vi "CIF_Iceoryx_String_Tag Update Test Cases.vi"() -> (0 "error out":errorcluster, 2 "status":string, 3 "pass":bool)   [LabVIEW 2021]
uses:
  CIF_Iceoryx_Chn_String.lvclass
  D:/dev/Packages/CIF_Channels_Core/src/Iceorxy_Channels/CIF_Iceoryx_BB/CIF_Iceoryx_BB.lvclass
  D:/dev/Packages/CIF_Channels_Core/src/CIFChannels/CIFChannels.lvclass
  ChannelCommon/typedef/Direction.ctl
  ChannelCommon/typedef/New FIFO Instance Response.ctl
  CIFChannels/CIFChannels.lvclass/CIFChannels.ctl
  ChannelCommon/typedef/New FIFO Config.ctl
  ChannelCommon/typedef/FIFO Flags.ctl
  ChannelCommon/ChannelCommon.lvlib
  CIFChannels/CIFChannels.lvclass
  <vilib>/CIF Foundation/CIF Iceoryx/Iceoryx.lvlib
  CIF_Iceoryx_BB/CIF_Iceoryx_BB.lvclass
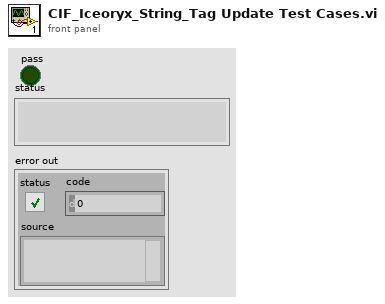
[diagram p1: front panel]
types:
  T1 = typedef "ChannelCommon.lvlib/Direction.ctl" = enum8{"Publisher", "Subscriber"}
  T2 = typedef "ChannelCommon.lvlib/New FIFO Instance Response.ctl" = cluster{"Publisher":string, "Custom Data":u8[]}
  T3 = typedef "ChannelCommon.lvlib/New FIFO Config.ctl" = cluster{"Max Bytes/Msg":u64, "Max Msg/FIFO":u64, "FIFO Flags":T4, "Best Effort Subscribers":u32, "Backpressure Subscribers":u32}
  T4 = typedef "ChannelCommon.lvlib/FIFO Flags.ctl" = cluster{"Backpressure":bool, "Extended Config":bool}
  T5 = typedef "Iceoryx.lvlib/BB Refnum.ctl" = cluster{"refnum":u64, "BB":enum8{"bb"}}
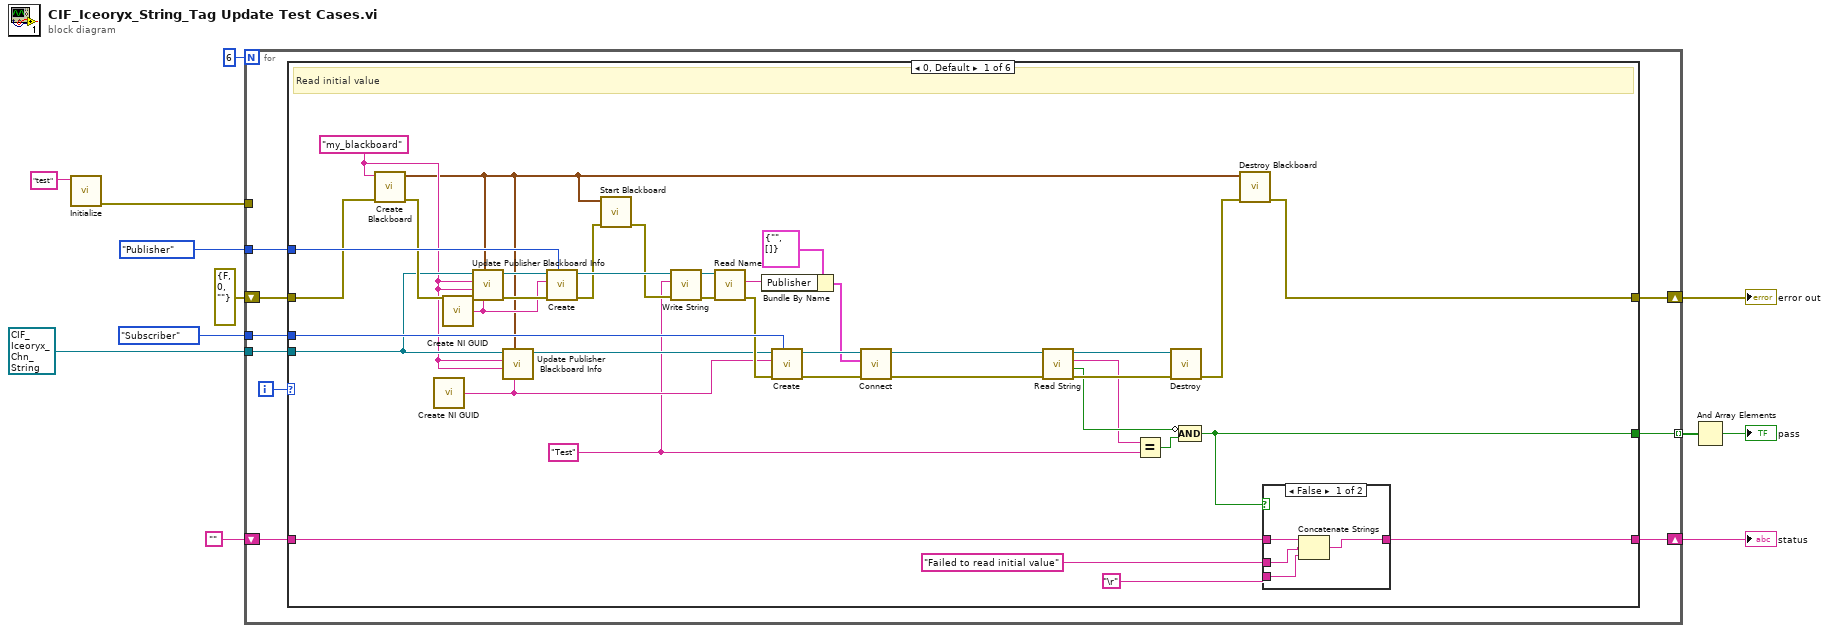
[diagram p0: block diagram]
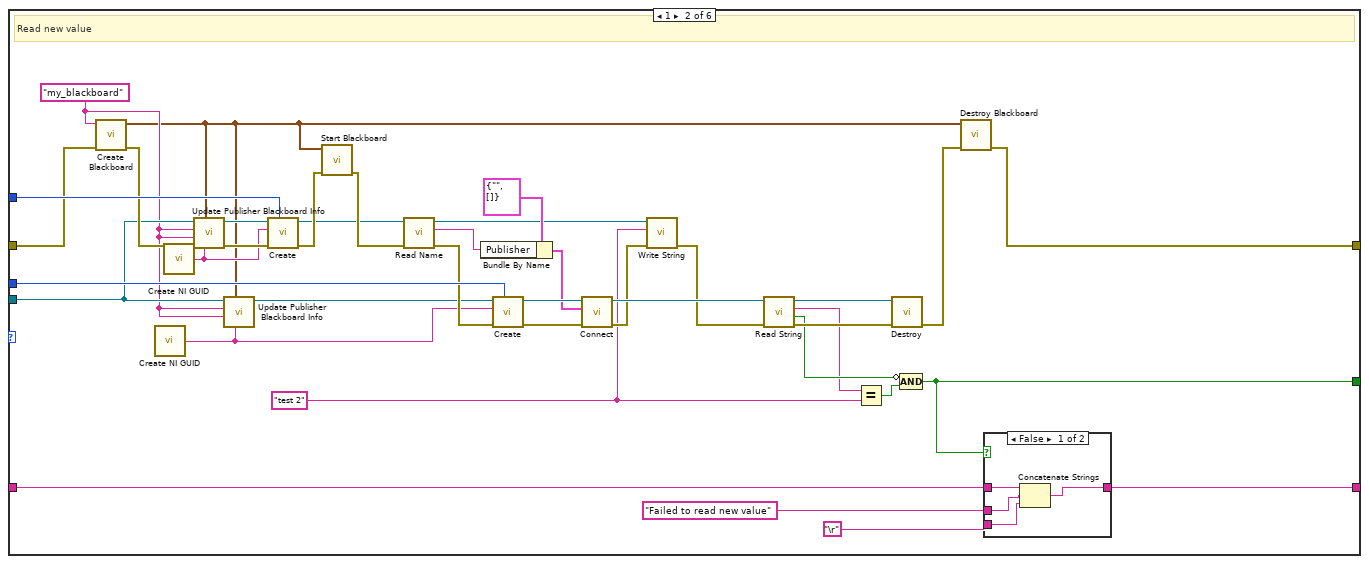
[diagram p3: hidden frame]
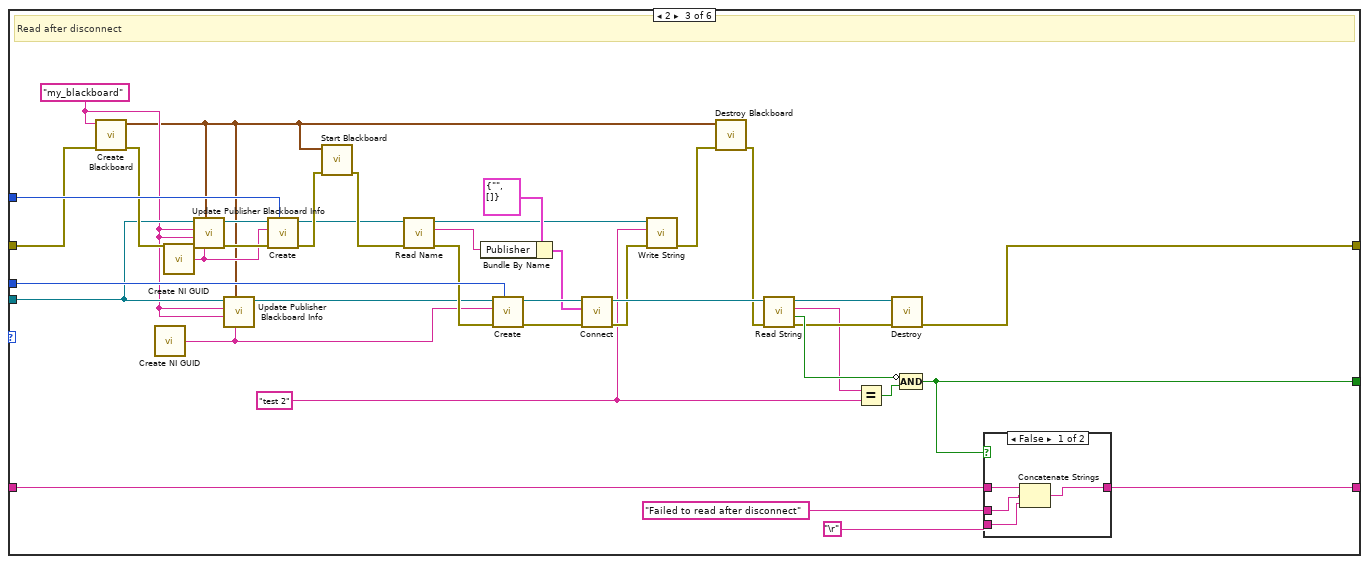
[diagram p5: hidden frame]
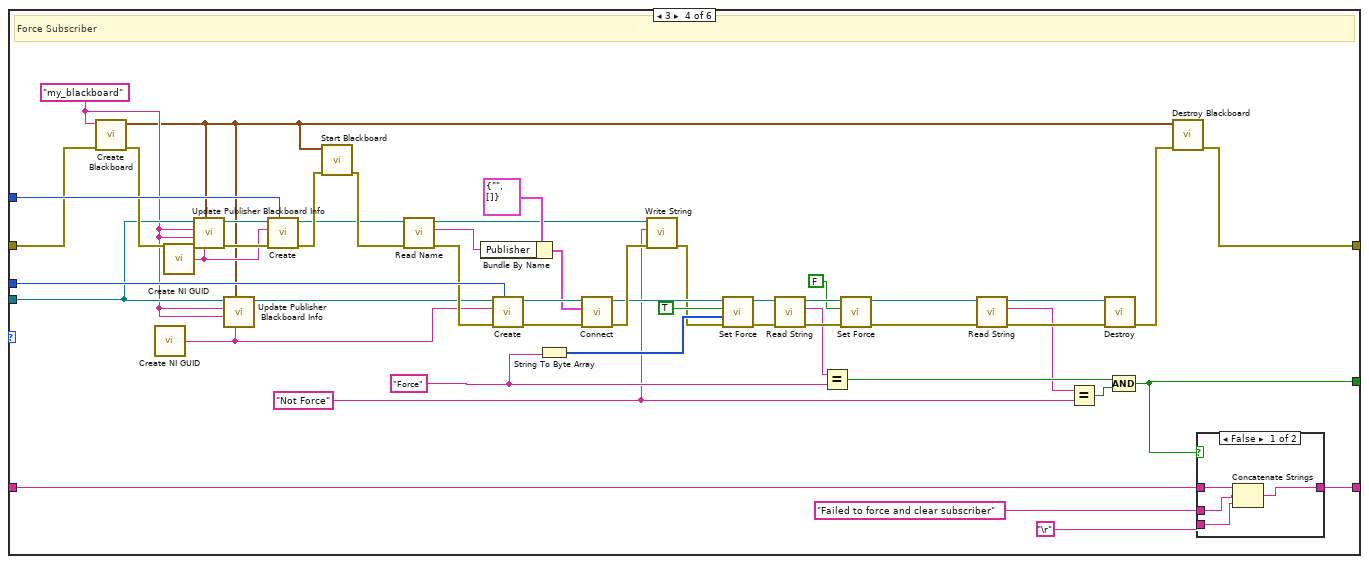
[diagram p7: hidden frame]
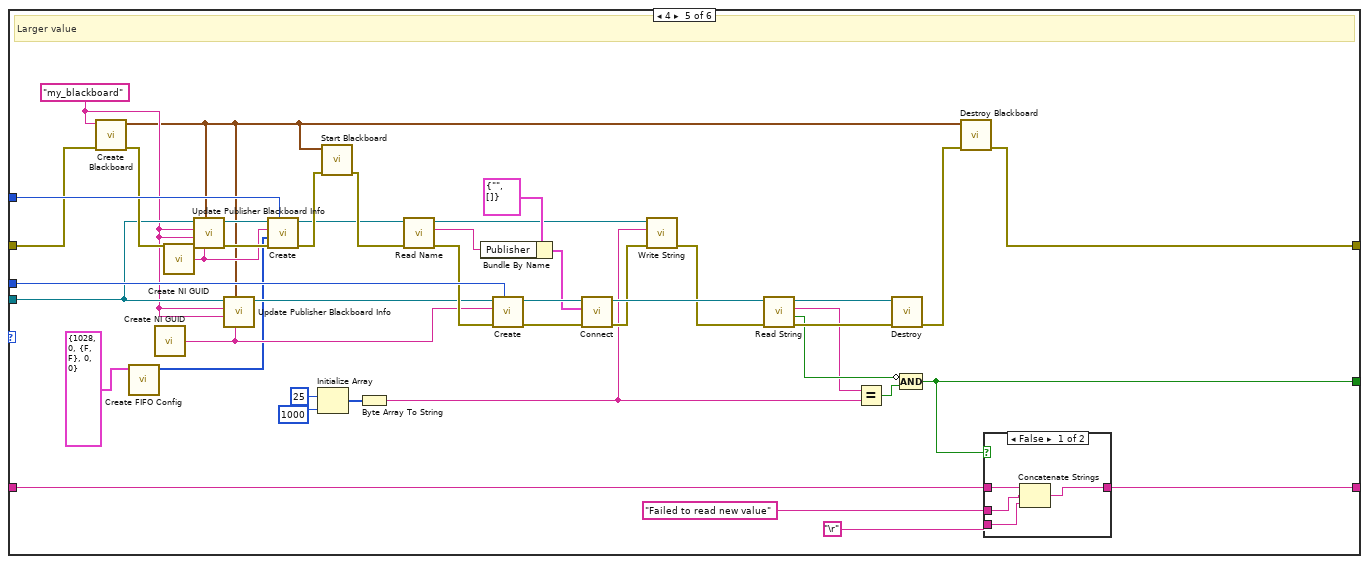
[diagram p9: hidden frame]
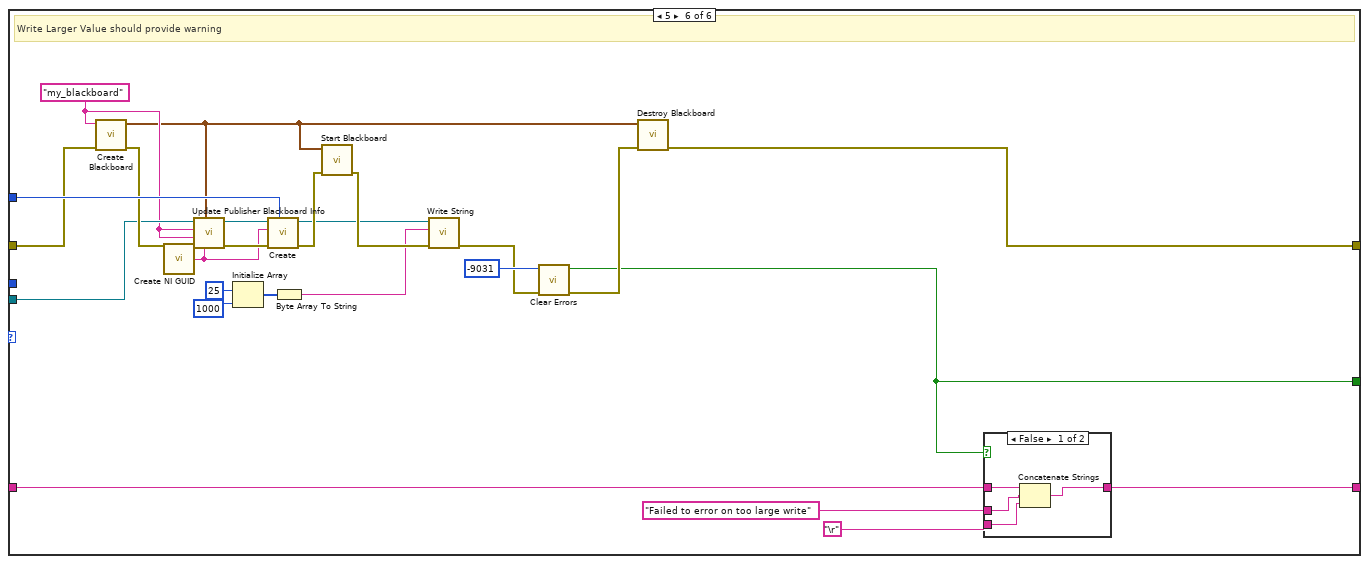
[diagram p11: hidden frame]
diagram:
  n1 = call <vilib>:"Initialize.vi"("Node name"="test") -> ("error out"=w6:errorcluster)  [unwired: 10 in]
  n2 = for {
    N: 6 -> [_]
    tunnel: [w21] -> w12 mode=indexing
    shift-right: [w19] -> w3
    shift-left: errorcluster {"status"=FALSE, "code"=0, "source"=""} ("error out") -> [w20]
    shift-right: [w16] -> w1
    shift-left: "" -> [w17]
    tunnel: refnum<class "CIF_Iceoryx_Chn_String.lvclass"> refnum ("CIF_CIPC_Chn_String.lvclass") -> [w15]
    tunnel: Direction."Publisher" ("Direction") -> [w14]
    tunnel: Direction."Subscriber" ("Direction") -> [w13]
    tunnel: w6 -> [_]
    i -> [w18]
    n3 = case shown="0, Default" w18 {
      tunnel: [w49 w92 w136 w191 w237 w253] -> w21
      tunnel: w20 -> [w42 w86 w130 w186 w231 w272]
      tunnel: [w35 w80 w110 w180 w225 w267] -> w19
      tunnel: w17 -> [w59 w102 w145 w199 w247 w277]
      tunnel: [w58 w101 w144 w198 w246 w276] -> w16
      tunnel: w15 -> [w28 w76 w122 w176 w221 w265]
      tunnel: w14 -> [w47 w90 w134 w190 w235 w273]
      tunnel: w13 -> [w46 w89 w133 w189 w234 _]
      frame 0, Default {
        w23 = "Test"
        w26 = "my_blackboard" ("Blackboard name")
        # "Read initial value"
        n4 = call <vilib>:"Create Blackboard.vi"("error in (no error)"=w42, "Blackboard name"=w26) -> ("error out"=w39:errorcluster, "Blackboard Reference"=w24:T5)  [unwired: 8 in]
        n5 = call <vilib>:"Create NI GUID.vi"() -> ("NI GUID"=w25:string)
        n6 = call <vilib>:"Create NI GUID.vi"() -> ("NI GUID"=w33:string)
        n7 = call "Update Publisher Blackboard Info.vi"("Topic"=w33, "Blackboard Reference"=w24, "error in (no error)"=w39, "Blackboard name"=w26, "Plugin name"=w26, "CIF_Iceoryx_BB in"=w28) -> ("error out"=w38:errorcluster, "CIF_Iceoryx_BB out"=w37:refnum<class "CIF_Iceoryx_Chn_String.lvclass">)  [unwired: 3 in, 1 out]
        n8 = call "Update Publisher Blackboard Info.vi"("Topic"=w25, "Blackboard Reference"=w24, "Blackboard name"=w26, "Plugin name"=w26, "CIF_Iceoryx_BB in"=w28) -> ("CIF_Iceoryx_BB out"=w27:refnum<class "CIF_Iceoryx_Chn_String.lvclass">)  [unwired: 4 in, 2 out]
        n9 = call-dynamic "Create.vi"("Direction"=w47, "error in (no error)"=w38, "Name"=w33, "CIFTag in"=w37) -> ("error out"=w41:errorcluster, "CIFTag out"=w45:refnum<class "CIF_Iceoryx_Chn_String.lvclass">)  [unwired: 6 in]
        n10 = call <vilib>:"Start Blackboard.vi"("error in (no error)"=w41, "Blackboard Reference"=w24) -> ("error out"=w40:errorcluster)  [unwired: 9 in]
        n11 = call-dynamic "Write String.vi"("error in (no error)"=w40, "Data"=w23, "CIFTag in"=w45) -> ("error out"=w32:errorcluster, "CIFTag out"=w31:refnum<class "CIF_Iceoryx_Chn_String.lvclass">)  [unwired: 6 in, 1 out]
        n12 = call "Read Name.vi"("error in (no error)"=w32, "CIFChannels in"=w31) -> ("error out"=w29:errorcluster, "Name"=w30:string)  [unwired: 7 in, 1 out]
        n13 = Bundle By Name(cluster=T2 {"Publisher"="", "Custom Data"=[]} ("Connection"), "Publisher"=w30) -> (w43:T2)
        n14 = call-dynamic "Create.vi"("Direction"=w46, "error in (no error)"=w29, "Name"=w25, "CIFTag in"=w27) -> ("error out"=w54:errorcluster, "CIFTag out"=w55:refnum<class "CIF_Iceoryx_Chn_String.lvclass">)  [unwired: 6 in]
        n15 = call-dynamic "Connect.vi"("error in (no error)"=w54, "Connection"=w43, "CIF_Iceoryx_BB"=w55) -> ("error out"=w34:errorcluster, "CIF_Iceoryx_BB"=w53:refnum<class "CIF_Iceoryx_Chn_String.lvclass">)  [unwired: 7 in]
        n16 = call-dynamic "Read String.vi"("error in (no error)"=w34, "CIFTag in"=w53) -> ("error out"=w51:errorcluster, "timed out?"=w48:bool, "Data"=w22:string, "CIFTag out"=w52:refnum<class "CIF_Iceoryx_Chn_String.lvclass">)  [unwired: 6 in]
        n17 = Equal?(x=w22, y=w23) -> (x = y?=w50:bool)
        n18 = call-dynamic "Destroy.vi"("error in (no error)"=w51, "CIF_Iceoryx_BB in"=w52) -> ("error out"=w36:errorcluster)  [unwired: 8 in, 1 out]
        n19 = Compound Arithmetic op=AND(invert w48, w50) -> (w49:bool)
        n20 = call <vilib>:"Destroy Blackboard.vi"("error in (no error)"=w36, "Blackboard Reference"=w24) -> ("error out"=w35:errorcluster)  [unwired: 8 in, 1 out]
        n21 = case shown="False" w49 {
          tunnel: w59 -> [w63 w64]
          tunnel: [w60 w64] -> w58
          tunnel: "Failed to read initial value" -> [w62 _]
          tunnel: "\r" -> [w61 _]
          frame False {
            n22 = Concatenate Strings(w63, w62, w61) -> (w60:string)
          }
          frame True {
          }
        }
      }
      frame 1 {
        w66 = "test 2" ("Data")
        w74 = "my_blackboard" ("Blackboard name")
        # "Read new value"
        n23 = call <vilib>:"Create Blackboard.vi"("error in (no error)"=w86, "Blackboard name"=w74) -> ("error out"=w84:errorcluster, "Blackboard Reference"=w72:T5)  [unwired: 8 in]
        n24 = call <vilib>:"Create NI GUID.vi"() -> ("NI GUID"=w73:string)
        n25 = call <vilib>:"Create NI GUID.vi"() -> ("NI GUID"=w79:string)
        n26 = call "Update Publisher Blackboard Info.vi"("Topic"=w79, "Blackboard Reference"=w72, "error in (no error)"=w84, "Blackboard name"=w74, "Plugin name"=w74, "CIF_Iceoryx_BB in"=w76) -> ("error out"=w83:errorcluster, "CIF_Iceoryx_BB out"=w82:refnum<class "CIF_Iceoryx_Chn_String.lvclass">)  [unwired: 3 in, 1 out]
        n27 = call "Update Publisher Blackboard Info.vi"("Topic"=w73, "Blackboard Reference"=w72, "Blackboard name"=w74, "Plugin name"=w74, "CIF_Iceoryx_BB in"=w76) -> ("CIF_Iceoryx_BB out"=w75:refnum<class "CIF_Iceoryx_Chn_String.lvclass">)  [unwired: 4 in, 2 out]
        n28 = call-dynamic "Create.vi"("Direction"=w90, "error in (no error)"=w83, "Name"=w79, "CIFTag in"=w82) -> ("error out"=w85:errorcluster, "CIFTag out"=w69:refnum<class "CIF_Iceoryx_Chn_String.lvclass">)  [unwired: 6 in]
        n29 = call <vilib>:"Start Blackboard.vi"("error in (no error)"=w85, "Blackboard Reference"=w72) -> ("error out"=w70:errorcluster)  [unwired: 9 in]
        n30 = call "Read Name.vi"("error in (no error)"=w70, "CIFChannels in"=w69) -> ("error out"=w77:errorcluster, "Name"=w78:string, "CIFChannels out"=w71:refnum<class "CIF_Iceoryx_Chn_String.lvclass">)  [unwired: 7 in]
        n31 = Bundle By Name(cluster=T2 {"Publisher"="", "Custom Data"=[]} ("Connection"), "Publisher"=w78) -> (w87:T2)
        n32 = call-dynamic "Create.vi"("Direction"=w89, "error in (no error)"=w77, "Name"=w73, "CIFTag in"=w75) -> ("error out"=w97:errorcluster, "CIFTag out"=w98:refnum<class "CIF_Iceoryx_Chn_String.lvclass">)  [unwired: 6 in]
        n33 = call-dynamic "Connect.vi"("error in (no error)"=w97, "Connection"=w87, "CIF_Iceoryx_BB"=w98) -> ("error out"=w68:errorcluster, "CIF_Iceoryx_BB"=w96:refnum<class "CIF_Iceoryx_Chn_String.lvclass">)  [unwired: 7 in]
        n34 = call-dynamic "Write String.vi"("error in (no error)"=w68, "Data"=w66, "CIFTag in"=w71) -> ("error out"=w67:errorcluster)  [unwired: 6 in, 2 out]
        n35 = call-dynamic "Read String.vi"("error in (no error)"=w67, "CIFTag in"=w96) -> ("error out"=w94:errorcluster, "timed out?"=w91:bool, "Data"=w65:string, "CIFTag out"=w95:refnum<class "CIF_Iceoryx_Chn_String.lvclass">)  [unwired: 6 in]
        n36 = Equal?(x=w65, y=w66) -> (x = y?=w93:bool)
        n37 = call-dynamic "Destroy.vi"("error in (no error)"=w94, "CIF_Iceoryx_BB in"=w95) -> ("error out"=w81:errorcluster)  [unwired: 8 in, 1 out]
        n38 = Compound Arithmetic op=AND(invert w91, w93) -> (w92:bool)
        n39 = call <vilib>:"Destroy Blackboard.vi"("error in (no error)"=w81, "Blackboard Reference"=w72) -> ("error out"=w80:errorcluster)  [unwired: 8 in, 1 out]
        n40 = case shown="False" w92 {
          tunnel: w102 -> [w106 w107]
          tunnel: [w103 w107] -> w101
          tunnel: "Failed to read new value" -> [w105 _]
          tunnel: "\r" -> [w104 _]
          frame False {
            n41 = Concatenate Strings(w106, w105, w104) -> (w103:string)
          }
          frame True {
          }
        }
      }
      frame 2 {
        w108 = "test 2" ("Data")
        w120 = "my_blackboard" ("Blackboard name")
        # "Read after disconnect"
        n42 = call <vilib>:"Create Blackboard.vi"("error in (no error)"=w130, "Blackboard name"=w120) -> ("error out"=w128:errorcluster, "Blackboard Reference"=w118:T5)  [unwired: 8 in]
        n43 = call <vilib>:"Create NI GUID.vi"() -> ("NI GUID"=w119:string)
        n44 = call <vilib>:"Create NI GUID.vi"() -> ("NI GUID"=w125:string)
        n45 = call "Update Publisher Blackboard Info.vi"("Topic"=w125, "Blackboard Reference"=w118, "error in (no error)"=w128, "Blackboard name"=w120, "Plugin name"=w120, "CIF_Iceoryx_BB in"=w122) -> ("error out"=w127:errorcluster, "CIF_Iceoryx_BB out"=w126:refnum<class "CIF_Iceoryx_Chn_String.lvclass">)  [unwired: 3 in, 1 out]
        n46 = call "Update Publisher Blackboard Info.vi"("Topic"=w119, "Blackboard Reference"=w118, "Blackboard name"=w120, "Plugin name"=w120, "CIF_Iceoryx_BB in"=w122) -> ("CIF_Iceoryx_BB out"=w121:refnum<class "CIF_Iceoryx_Chn_String.lvclass">)  [unwired: 4 in, 2 out]
        n47 = call-dynamic "Create.vi"("Direction"=w134, "error in (no error)"=w127, "Name"=w125, "CIFTag in"=w126) -> ("error out"=w129:errorcluster, "CIFTag out"=w115:refnum<class "CIF_Iceoryx_Chn_String.lvclass">)  [unwired: 6 in]
        n48 = call <vilib>:"Start Blackboard.vi"("error in (no error)"=w129, "Blackboard Reference"=w118) -> ("error out"=w116:errorcluster)  [unwired: 9 in]
        n49 = call "Read Name.vi"("error in (no error)"=w116, "CIFChannels in"=w115) -> ("error out"=w123:errorcluster, "Name"=w124:string, "CIFChannels out"=w117:refnum<class "CIF_Iceoryx_Chn_String.lvclass">)  [unwired: 7 in]
        n50 = Bundle By Name(cluster=T2 {"Publisher"="", "Custom Data"=[]} ("Connection"), "Publisher"=w124) -> (w131:T2)
        n51 = call-dynamic "Create.vi"("Direction"=w133, "error in (no error)"=w123, "Name"=w119, "CIFTag in"=w121) -> ("error out"=w140:errorcluster, "CIFTag out"=w141:refnum<class "CIF_Iceoryx_Chn_String.lvclass">)  [unwired: 6 in]
        n52 = call-dynamic "Connect.vi"("error in (no error)"=w140, "Connection"=w131, "CIF_Iceoryx_BB"=w141) -> ("error out"=w114:errorcluster, "CIF_Iceoryx_BB"=w139:refnum<class "CIF_Iceoryx_Chn_String.lvclass">)  [unwired: 7 in]
        n53 = call-dynamic "Write String.vi"("error in (no error)"=w114, "Data"=w108, "CIFTag in"=w117) -> ("error out"=w112:errorcluster)  [unwired: 6 in, 2 out]
        n54 = call <vilib>:"Destroy Blackboard.vi"("error in (no error)"=w112, "Blackboard Reference"=w118) -> ("error out"=w111:errorcluster)  [unwired: 8 in, 1 out]
        n55 = call-dynamic "Read String.vi"("error in (no error)"=w111, "CIFTag in"=w139) -> ("error out"=w113:errorcluster, "timed out?"=w135:bool, "Data"=w109:string, "CIFTag out"=w138:refnum<class "CIF_Iceoryx_Chn_String.lvclass">)  [unwired: 6 in]
        n56 = Equal?(x=w109, y=w108) -> (x = y?=w137:bool)
        n57 = call-dynamic "Destroy.vi"("error in (no error)"=w113, "CIF_Iceoryx_BB in"=w138) -> ("error out"=w110:errorcluster)  [unwired: 8 in, 1 out]
        n58 = Compound Arithmetic op=AND(invert w135, w137) -> (w136:bool)
        n59 = case shown="False" w136 {
          tunnel: w145 -> [w149 w150]
          tunnel: [w146 w150] -> w144
          tunnel: "Failed to read after disconnect" -> [w148 _]
          tunnel: "\r" -> [w147 _]
          frame False {
            n60 = Concatenate Strings(w149, w148, w147) -> (w146:string)
          }
          frame True {
          }
        }
      }
      frame 3 {
        w151 = "Not Force" ("Data")
        w154 = "Force" ("string")
        w174 = "my_blackboard" ("Blackboard name")
        # "Force Subscriber"
        n61 = call <vilib>:"Create Blackboard.vi"("error in (no error)"=w186, "Blackboard name"=w174) -> ("error out"=w184:errorcluster, "Blackboard Reference"=w172:T5)  [unwired: 8 in]
        n62 = call <vilib>:"Create NI GUID.vi"() -> ("NI GUID"=w173:string)
        n63 = call <vilib>:"Create NI GUID.vi"() -> ("NI GUID"=w179:string)
        n64 = call "Update Publisher Blackboard Info.vi"("Topic"=w179, "Blackboard Reference"=w172, "error in (no error)"=w184, "Blackboard name"=w174, "Plugin name"=w174, "CIF_Iceoryx_BB in"=w176) -> ("error out"=w183:errorcluster, "CIF_Iceoryx_BB out"=w182:refnum<class "CIF_Iceoryx_Chn_String.lvclass">)  [unwired: 3 in, 1 out]
        n65 = call "Update Publisher Blackboard Info.vi"("Topic"=w173, "Blackboard Reference"=w172, "Blackboard name"=w174, "Plugin name"=w174, "CIF_Iceoryx_BB in"=w176) -> ("CIF_Iceoryx_BB out"=w175:refnum<class "CIF_Iceoryx_Chn_String.lvclass">)  [unwired: 4 in, 2 out]
        n66 = call-dynamic "Create.vi"("Direction"=w190, "error in (no error)"=w183, "Name"=w179, "CIFTag in"=w182) -> ("error out"=w185:errorcluster, "CIFTag out"=w169:refnum<class "CIF_Iceoryx_Chn_String.lvclass">)  [unwired: 6 in]
        n67 = call <vilib>:"Start Blackboard.vi"("error in (no error)"=w185, "Blackboard Reference"=w172) -> ("error out"=w170:errorcluster)  [unwired: 9 in]
        n68 = call "Read Name.vi"("error in (no error)"=w170, "CIFChannels in"=w169) -> ("error out"=w177:errorcluster, "Name"=w178:string, "CIFChannels out"=w171:refnum<class "CIF_Iceoryx_Chn_String.lvclass">)  [unwired: 7 in]
        n69 = Bundle By Name(cluster=T2 {"Publisher"="", "Custom Data"=[]} ("Connection"), "Publisher"=w178) -> (w187:T2)
        n70 = call-dynamic "Create.vi"("Direction"=w189, "error in (no error)"=w177, "Name"=w173, "CIFTag in"=w175) -> ("error out"=w194:errorcluster, "CIFTag out"=w195:refnum<class "CIF_Iceoryx_Chn_String.lvclass">)  [unwired: 6 in]
        n71 = String To Byte Array(string=w154) -> (unsigned byte array=w167:u8[])
        n72 = call-dynamic "Connect.vi"("error in (no error)"=w194, "Connection"=w187, "CIF_Iceoryx_BB"=w195) -> ("error out"=w168:errorcluster, "CIF_Iceoryx_BB"=w165:refnum<class "CIF_Iceoryx_Chn_String.lvclass">)  [unwired: 7 in]
        n73 = call-dynamic "Write String.vi"("error in (no error)"=w168, "Data"=w151, "CIFTag in"=w171) -> ("error out"=w158:errorcluster)  [unwired: 6 in, 2 out]
        n74 = call "Set Force.vi"("error in (no error)"=w158, "Force Data"=w167, "Force Active"=TRUE, "CIFChannels in"=w165) -> ("error out"=w163:errorcluster, "CIFChannels out"=w164:refnum<class "CIF_Iceoryx_Chn_String.lvclass">)  [unwired: 6 in]
        n75 = call-dynamic "Read String.vi"("error in (no error)"=w163, "CIFTag in"=w164) -> ("error out"=w161:errorcluster, "Data"=w153:string, "CIFTag out"=w162:refnum<class "CIF_Iceoryx_Chn_String.lvclass">)  [unwired: 6 in, 1 out]
        n76 = Equal?(x=w153, y=w154) -> (x = y?=w155:bool)
        n77 = call "Set Force.vi"("error in (no error)"=w161, "Force Active"=FALSE, "CIFChannels in"=w162) -> ("error out"=w157:errorcluster, "CIFChannels out"=w159:refnum<class "CIF_Iceoryx_Chn_String.lvclass">)  [unwired: 7 in]
        n78 = call-dynamic "Read String.vi"("error in (no error)"=w157, "CIFTag in"=w159) -> ("error out"=w192:errorcluster, "Data"=w152:string, "CIFTag out"=w193:refnum<class "CIF_Iceoryx_Chn_String.lvclass">)  [unwired: 6 in, 1 out]
        n79 = Equal?(x=w152, y=w151) -> (x = y?=w156:bool)
        n80 = call-dynamic "Destroy.vi"("error in (no error)"=w192, "CIF_Iceoryx_BB in"=w193) -> ("error out"=w181:errorcluster)  [unwired: 8 in, 1 out]
        n81 = Compound Arithmetic op=AND(w155, w156) -> (w191:bool)
        n82 = call <vilib>:"Destroy Blackboard.vi"("error in (no error)"=w181, "Blackboard Reference"=w172) -> ("error out"=w180:errorcluster)  [unwired: 8 in, 1 out]
        n83 = case shown="False" w191 {
          tunnel: w199 -> [w203 w204]
          tunnel: [w200 w204] -> w198
          tunnel: "Failed to force and clear subscriber" -> [w202 _]
          tunnel: "\r" -> [w201 _]
          frame False {
            n84 = Concatenate Strings(w203, w202, w201) -> (w200:string)
          }
          frame True {
          }
        }
      }
      frame 4 {
        w219 = "my_blackboard" ("Blackboard name")
        # "Larger value"
        n85 = call <vilib>:"Create Blackboard.vi"("error in (no error)"=w231, "Blackboard name"=w219) -> ("error out"=w229:errorcluster, "Blackboard Reference"=w217:T5)  [unwired: 8 in]
        n86 = call "Create FIFO Config.vi"("New FIFO Config"=T3 {"Max Bytes/Msg"=1028, "Max Msg/FIFO"=0, "FIFO Flags"={"Backpressure"=FALSE, "Extended Config"=FALSE}, "Best Effort Subscribers"=0, "Backpressure Subscribers"=0}) -> ("Flattened FIFO Config"=w209:u8[])  [unwired: 10 in]
        n87 = call <vilib>:"Create NI GUID.vi"() -> ("NI GUID"=w218:string)
        n88 = call <vilib>:"Create NI GUID.vi"() -> ("NI GUID"=w224:string)
        n89 = call "Update Publisher Blackboard Info.vi"("Topic"=w224, "Blackboard Reference"=w217, "error in (no error)"=w229, "Blackboard name"=w219, "Plugin name"=w219, "CIF_Iceoryx_BB in"=w221) -> ("error out"=w228:errorcluster, "CIF_Iceoryx_BB out"=w227:refnum<class "CIF_Iceoryx_Chn_String.lvclass">)  [unwired: 3 in, 1 out]
        n90 = call "Update Publisher Blackboard Info.vi"("Topic"=w218, "Blackboard Reference"=w217, "Blackboard name"=w219, "Plugin name"=w219, "CIF_Iceoryx_BB in"=w221) -> ("CIF_Iceoryx_BB out"=w220:refnum<class "CIF_Iceoryx_Chn_String.lvclass">)  [unwired: 4 in, 2 out]
        n91 = call-dynamic "Create.vi"("Direction"=w235, "error in (no error)"=w228, "Custom Config Data"=w209, "Name"=w224, "CIFTag in"=w227) -> ("error out"=w230:errorcluster, "CIFTag out"=w214:refnum<class "CIF_Iceoryx_Chn_String.lvclass">)  [unwired: 5 in]
        n92 = Initialize Array(u8 25 ("element"), 1000 ("dimension size")) -> (w208:u8[])
        n93 = call <vilib>:"Start Blackboard.vi"("error in (no error)"=w230, "Blackboard Reference"=w217) -> ("error out"=w215:errorcluster)  [unwired: 9 in]
        n94 = Byte Array To String(unsigned byte array=w208) -> (string=w205:string)
        n95 = call "Read Name.vi"("error in (no error)"=w215, "CIFChannels in"=w214) -> ("error out"=w222:errorcluster, "Name"=w223:string, "CIFChannels out"=w216:refnum<class "CIF_Iceoryx_Chn_String.lvclass">)  [unwired: 7 in]
        n96 = Bundle By Name(cluster=T2 {"Publisher"="", "Custom Data"=[]} ("Connection"), "Publisher"=w223) -> (w232:T2)
        n97 = call-dynamic "Create.vi"("Direction"=w234, "error in (no error)"=w222, "Name"=w218, "CIFTag in"=w220) -> ("error out"=w242:errorcluster, "CIFTag out"=w243:refnum<class "CIF_Iceoryx_Chn_String.lvclass">)  [unwired: 6 in]
        n98 = call-dynamic "Connect.vi"("error in (no error)"=w242, "Connection"=w232, "CIF_Iceoryx_BB"=w243) -> ("error out"=w213:errorcluster, "CIF_Iceoryx_BB"=w241:refnum<class "CIF_Iceoryx_Chn_String.lvclass">)  [unwired: 7 in]
        n99 = call-dynamic "Write String.vi"("error in (no error)"=w213, "Data"=w205, "CIFTag in"=w216) -> ("error out"=w212:errorcluster)  [unwired: 6 in, 2 out]
        n100 = call-dynamic "Read String.vi"("error in (no error)"=w212, "CIFTag in"=w241) -> ("error out"=w239:errorcluster, "timed out?"=w236:bool, "Data"=w211:string, "CIFTag out"=w240:refnum<class "CIF_Iceoryx_Chn_String.lvclass">)  [unwired: 6 in]
        n101 = Equal?(x=w211, y=w205) -> (x = y?=w238:bool)
        n102 = call-dynamic "Destroy.vi"("error in (no error)"=w239, "CIF_Iceoryx_BB in"=w240) -> ("error out"=w226:errorcluster)  [unwired: 8 in, 1 out]
        n103 = Compound Arithmetic op=AND(invert w236, w238) -> (w237:bool)
        n104 = call <vilib>:"Destroy Blackboard.vi"("error in (no error)"=w226, "Blackboard Reference"=w217) -> ("error out"=w225:errorcluster)  [unwired: 8 in, 1 out]
        n105 = case shown="False" w237 {
          tunnel: w247 -> [w251 w252]
          tunnel: [w248 w252] -> w246
          tunnel: "Failed to read new value" -> [w250 _]
          tunnel: "\r" -> [w249 _]
          frame False {
            n106 = Concatenate Strings(w251, w250, w249) -> (w248:string)
          }
          frame True {
          }
        }
      }
      frame 5 {
        w264 = "my_blackboard" ("Blackboard name")
        # "Write Larger Value should provide warning"
        n107 = call <vilib>:"Create Blackboard.vi"("error in (no error)"=w272, "Blackboard name"=w264) -> ("error out"=w270:errorcluster, "Blackboard Reference"=w263:T5)  [unwired: 8 in]
        n108 = call <vilib>:"Create NI GUID.vi"() -> ("NI GUID"=w266:string)
        n109 = call "Update Publisher Blackboard Info.vi"("Topic"=w266, "Blackboard Reference"=w263, "error in (no error)"=w270, "Blackboard name"=w264, "Plugin name"=w264, "CIF_Iceoryx_BB in"=w265) -> ("error out"=w269:errorcluster, "CIF_Iceoryx_BB out"=w268:refnum<class "CIF_Iceoryx_Chn_String.lvclass">)  [unwired: 3 in, 1 out]
        n110 = Initialize Array(u8 25 ("element"), 1000 ("dimension size")) -> (w261:u8[])
        n111 = call-dynamic "Create.vi"("Direction"=w273, "error in (no error)"=w269, "Name"=w266, "CIFTag in"=w268) -> ("error out"=w271:errorcluster, "CIFTag out"=w258:refnum<class "CIF_Iceoryx_Chn_String.lvclass">)  [unwired: 6 in]
        n112 = Byte Array To String(unsigned byte array=w261) -> (string=w257:string)
        n113 = call <vilib>:"Start Blackboard.vi"("error in (no error)"=w271, "Blackboard Reference"=w263) -> ("error out"=w259:errorcluster)  [unwired: 9 in]
        n114 = call-dynamic "Write String.vi"("error in (no error)"=w259, "Data"=w257, "CIFTag in"=w258) -> ("error out"=w255:errorcluster)  [unwired: 6 in, 2 out]
        n115 = call <vilib>:"Clear Errors.vi"("error in (no error)"=w255, "specific error code to clear (0: all)"=-9031) -> ("error out"=w254:errorcluster, "specific error cleared?"=w253:bool)  [unwired: 4 in]
        n116 = call <vilib>:"Destroy Blackboard.vi"("error in (no error)"=w254, "Blackboard Reference"=w263) -> ("error out"=w267:errorcluster)  [unwired: 8 in, 1 out]
        n117 = case shown="False" w253 {
          tunnel: w277 -> [w281 w282]
          tunnel: [w278 w282] -> w276
          tunnel: "Failed to error on too large write" -> [w280 _]
          tunnel: "\r" -> [w279 _]
          frame False {
            n118 = Concatenate Strings(w281, w280, w279) -> (w278:string)
          }
          frame True {
          }
        }
      }
    }
  }
  "error out" <- w3
  "status" <- w1
  n119 = And Array Elements(Boolean array=w12) -> (logical AND=→"pass":bool)
